vi "Test Process Error in Process Loop Log Error Message.vi"(8 "error in (no error)":errorcluster, 11 "Test Case In":refnum<class "Logger Test.lvclass">) -> (0 "error out":errorcluster, 3 "Test Case Out":refnum<class "Logger Test.lvclass">)   [LabVIEW 2020, in "Logger Test.lvclass"]
uses:
  Logger Test.lvclass
  C:/Program Files (x86)/National Instruments/LabVIEW 2020/vi.lib/Astemes/LUnit/Test Case.lvclass
  source/Framework Test Suite/Mock Log Handler/Mock Log Handler.lvclass
  C:/git/astemes-triarc-framework/source/Framework/Logging/Logging.lvclass
  source/Framework Test Suite/Mock Process/Mock Process.lvclass
  C:/git/astemes-triarc-framework/source/Framework/Process/Process.lvclass
  source/Framework/Process/Process.lvclass/Process.ctl
  <vilib>/Astemes/LUnit/Test Case.lvclass/Test Case.ctl
  9649ef94-fae4-4853-88e7-0393d3ac6ac8.vi
  source/Framework/Process/Public/Lifecycle/Get Lifecycle State.vi
  source/Framework/Process/Protected/Messaging/Send Message.vi
  source/Framework/Process/Private/SubVIs/Wait for finish.vi
  source/Framework/Process/Private/SubVIs/Set Lifecycle State.vi
  <vilib>/Astemes/LUnit/Append Pass Result.vi
  <vilib>/Astemes/LUnit/Append Fail Result.vi
  <vilib>/Astemes/LUnit/Describe Comparison.vi
  <vilib>/Astemes/LUnit/Compare Variants.vi
  <vilib>/Utility/error.llb/Clear Errors.vi
  source/Framework/Process/Private/SubVIs/Handle Debug Data.vi
  <vilib>/Astemes/LUnit/Variant to string.vi
  source/Framework/Logging/Log Debug.vi
  <vilib>/AdvancedString/1D String Array to Delimited String.vi
  <vilib>/Utility/High Resolution Relative Seconds.vi
  source/Framework/Process/Public/Read Name.vi
  <vilib>/Utility/error.llb/Error Cluster From Error Code.vi
  <vilib>/Utility/Data Type/Get Type Information.vi
  <vilib>/Utility/LVClass/Get LV Class Name.vi
  source/Framework/Process/Process.lvclass
panel:
  out "Message":string
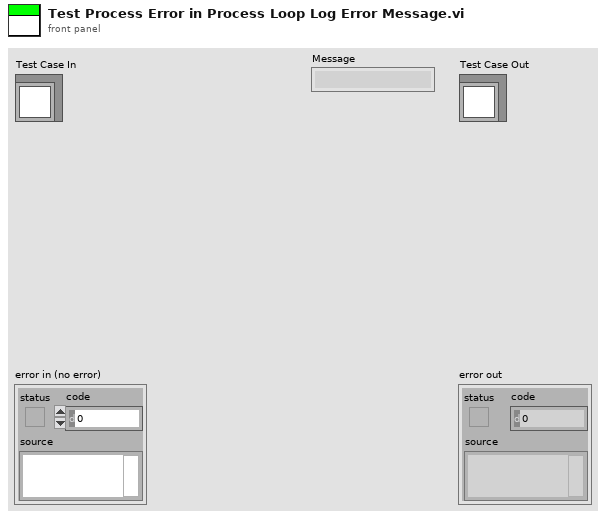
[diagram p1: front panel]
types:
  T1 = typedef "Mock Log Handler.lvclass/Log Entry.ctl" = cluster{"Level":string, "Source":string, "Message":string}
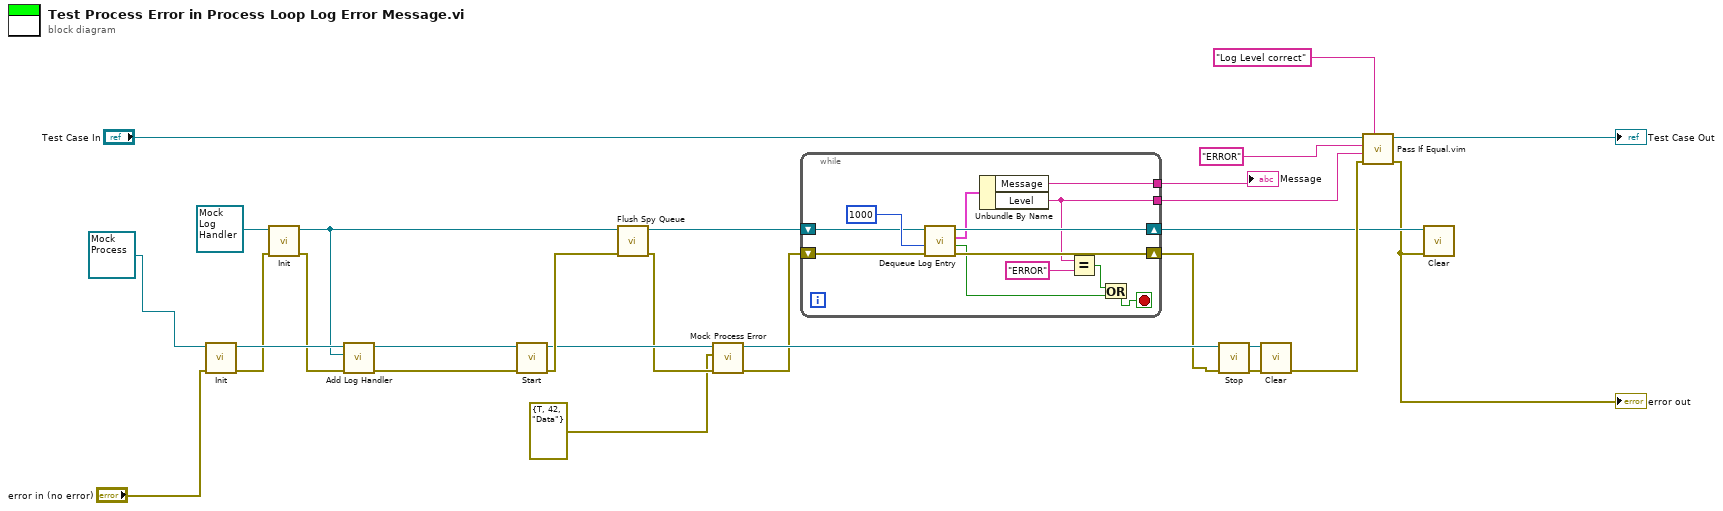
[diagram p0: block diagram]
diagram:
  n1 = call-dynamic "Init.vi"("error in (no error)"="error in (no error)", "Mock Process In"=refnum<class "Mock Process.lvclass"> refnum) -> ("error out"=w22:errorcluster, "Mock Process Out"=w25:refnum<class "Mock Process.lvclass">)  [unwired: 8 in]
  n2 = call-dynamic "Init.vi"("error in (no error)"=w22, "Mock Log Handler In"=refnum<class "Mock Log Handler.lvclass"> refnum ("Mock Log Handler.lvclass")) -> ("error out"=w21:errorcluster, "Mock Log Handler Out"=w14:refnum<class "Mock Log Handler.lvclass">)  [unwired: 8 in]
  n3 = call "Add Log Handler.vi"("error in (no error)"=w21, "Log Handler"=w14, "Process In"=w25) -> ("error out"=w17:errorcluster, "Process Out"=w10:refnum<class "Mock Process.lvclass">)  [unwired: 7 in]
  n4 = call "Start.vi"("error in (no error)"=w17, "Process In"=w10) -> ("error out"=w12:errorcluster, "Process Out"=w8:refnum<class "Mock Process.lvclass">)  [unwired: 7 in, 1 out]
  n5 = call "Flush Spy Queue.vi"("error in (no error)"=w12, "Mock Log Handler in"=w14) -> ("error out"=w6:errorcluster, "Mock Log Handler out"=w13:refnum<class "Mock Log Handler.lvclass">)  [unwired: 7 in, 1 out]
  n6 = call "Mock Process Error.vi"("error in (no error)"=w6, "Mock Error"=errorcluster {"status"=TRUE, "code"=42, "source"="Data"} ("error in (no error)"), "Mock Process in"=w8) -> ("error out"=w5:errorcluster, "Mock Process out"=w7:refnum<class "Mock Process.lvclass">)  [unwired: 7 in]
  n7 = while {
    tunnel: [w33] -> w19
    tunnel: [w34] -> w1
    shift-right: [w40] -> w20
    shift-left: w13 -> [w37]
    shift-right: [w35] -> w3
    shift-left: w5 -> [w36]
    stop <- w31 stop-if-true
    n8 = call "Dequeue Log Entry.vi"("error in (no error)"=w36, "timeout in ms (-1)"=1000, "Mock Log Handler in"=w37) -> ("error out"=w35:errorcluster, "timed out?"=w29:bool, "Entry"=w38:T1, "Mock Log Handler out"=w40:refnum<class "Mock Log Handler.lvclass">)  [unwired: 5 in]
    n9 = Unbundle By Name(w38) -> ("Message"=w34:string, "Level"=w33:string)
    n10 = Equal?(x=w33, y="ERROR") -> (x = y?=w30:bool)
    n11 = Or(x=w30, y=w29) -> (x .or. y?=w31:bool)
  }
  "Message" <- w1
  n12 = call "Stop.vi"("error in (no error)"=w3, "Process In"=w7) -> ("error out"=w16:errorcluster, "Process Out"=w15:refnum<class "Mock Process.lvclass">)  [unwired: 7 in, 1 out]
  n13 = call-dynamic "Clear.vi"("error in (no error)"=w16, "Mock Process In"=w15) -> ("error out"=w24:errorcluster)  [unwired: 9 in]
  n14 = call "Pass If Equal.vim"("Description"="Log Level correct", "error in (no error)"=w24, "Actual"=w19, "Expected"="ERROR", "LUnit Test Case In"="Test Case In") -> ("error out"=w2:errorcluster, "LUnit Test Case Out"=→"Test Case Out":refnum<class "Logger Test.lvclass">)  [unwired: 5 in]
  "error out" <- w2
  n15 = call-dynamic "Clear.vi"("error in (no error)"=w2, "Mock Log Handler In"=w20) -> ()  [unwired: 9 in, 1 out]
